vi "Run.vi"(8 "error in (no error)":errorcluster, 10 "UI Refs":T1, 11 "XY Plotter":refnum<class "XY Plotter.lvclass">) -> (0 "error out":errorcluster, 3 "XY Plotter out":refnum<class "XY Plotter.lvclass">)   [LabVIEW 2025, in "XY Plotter.lvlib" / "XY Plotter.lvclass"]
uses:
  XY Plotter.lvclass
  XY Plotter configuration/XY Plotter configuration.lvclass
  XY Plotter configuration/XY Plotter configuration.lvclass/XY Plotter configuration.ctl
  XY Plotter configuration/Read XY Plotter.vi
  Users/Public/Documents/Sandia National Labs/TSS Plugin/CEF.lvlibp/serializable configuration/CEF_serializable configuration.lvclass
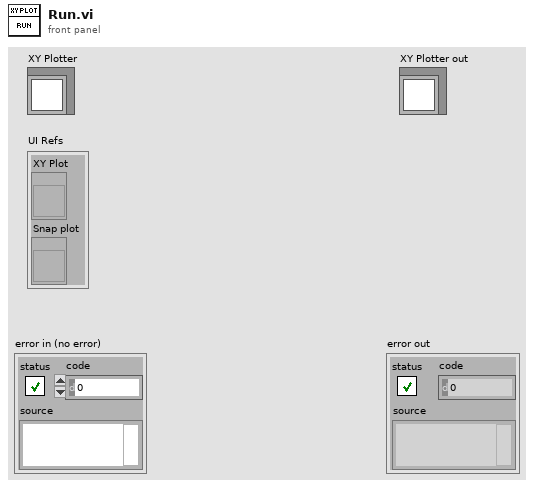
[diagram p1: front panel]
types:
  T1 = cluster{"XY Plot":refnum<vi>, "Snap plot":refnum<vi>}
  T2 = enum16{"Start Timer", "Read Time", "Pause", "Resume"}
  T3 = typedef "XY Plotter.lvlib/XY Plotter configuration.lvclass/XY Plotter.ctl" = cluster{"Data Rate":i32, "Y-Scales":cluster{"Label":string, "Max":dbl, "Min":dbl, "Unit":enum16{"---", "V", "mA", "sec", "dB", "deg", "in/s", "in", "lbf", "Hz", "psi", "gpm"}, "Visible":bool}[], "Note":string, "History Length":i32, "DataLog Path":path, "Plot type":bool, "X-Scales":cluster{"Label":string, "Max":dbl, "Min":dbl, "Unit":enum16{"---", "V", "mA", "sec", "dB", "deg", "in/s", "in", "lbf", "Hz", "psi", "gpm"}, "Visible":bool}[], "Plot List":cluster{"Plot Name":string, "X Scale Index":u32, "Y Scale Index":u32, "Visible":bool}[]}
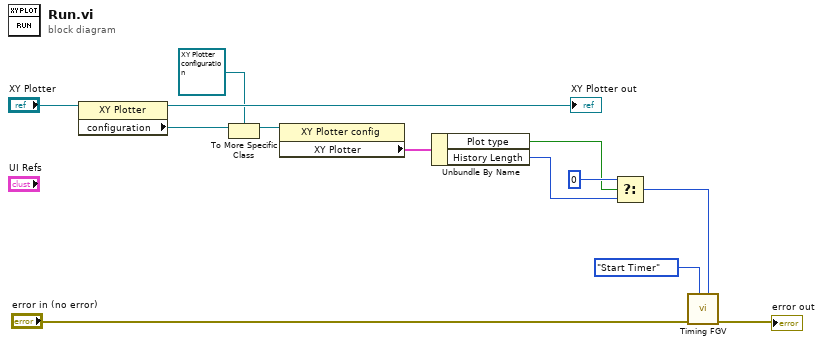
[diagram p0: block diagram]
diagram:
  n1 = property class="XY Plotter"(reference="XY Plotter") -> (reference out=→"XY Plotter out":refnum<class "XY Plotter.lvclass">, "configuration"=w12:refnum<class "CEF_serializable configuration.lvclass">)  [unwired: 1 in, 1 out]
  n2 = To More Specific Class(target class=refnum<class "XY Plotter configuration.lvclass"> refnum ("XY Plotter.lvlib:XY Plotter config"), reference=w12) -> (specific class reference=w13:refnum<class "XY Plotter configuration.lvclass">)  [unwired: 1 in, 1 out]
  n3 = property class="XY Plotter config"(reference=w13) -> ("XY Plotter"=w6:T3)  [unwired: 1 in, 2 out]
  n4 = Unbundle By Name(w6) -> ("Plot type"=w5:bool, "History Length"=w8:i32)
  n5 = Select(t=0 ("f"), s=w5, f=w8) -> (s? t:f=w2:i32)
  n6 = call "Timing FGV.vi"("Time Target (s)"=w2, "Timer Mode"=T2."Start Timer", "Error In"="error in (no error)") -> ("Error Out"=→"error out":errorcluster)  [unwired: 6 in, 2 out]
